vi "Feedback_ver1.vi"(4 "Default output":T3, 6 "Current Motion":T2, 7 "bound":dbl=10.0, 8 "Iteration":dbl, 9 "Sampled current position":dbl[](array[numeric]), 10 "Current Motion Output":T3, 11 "Initial constants":T4) -> (1 "Rawoffset":dbl[][](array[numeric]), 2 "Updated Motion Output Row":T1)   [LabVIEW 2019]
uses:
  Type_definition_current_motion.ctl
  Type_definition_updated_motion_output_row.ctl
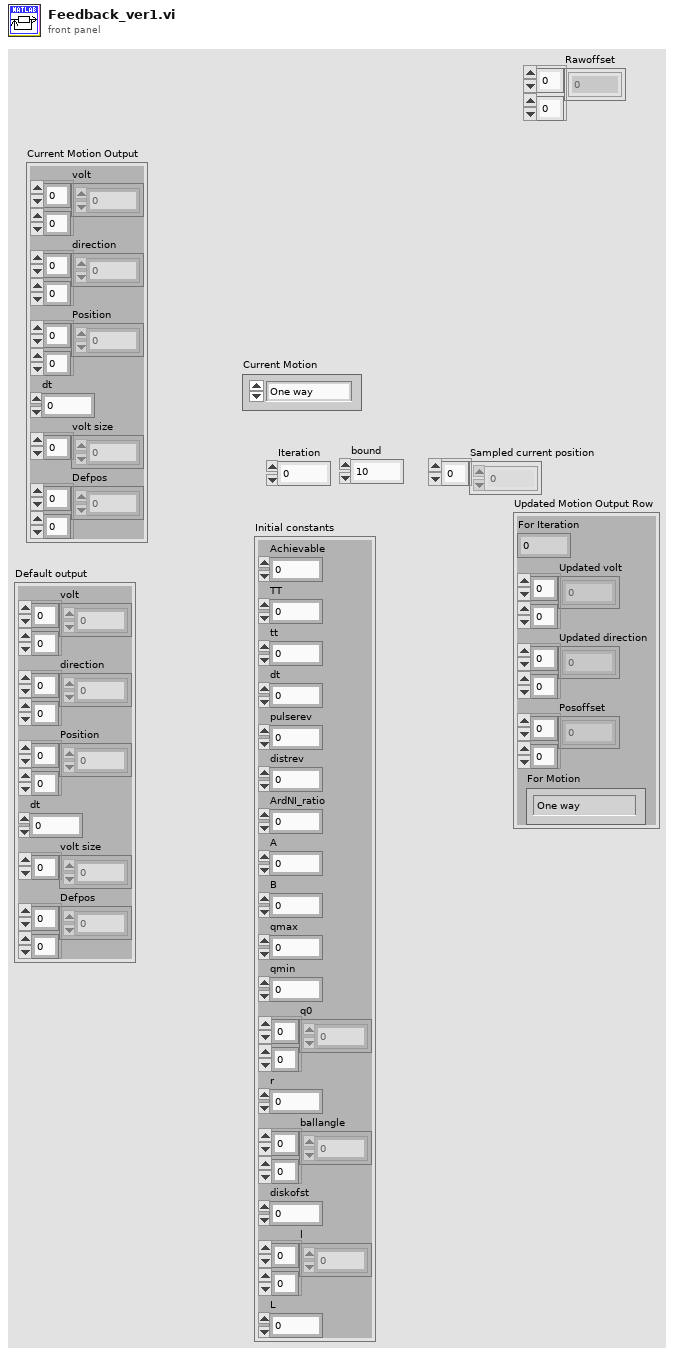
[diagram p1: front panel]
types:
  T1 = typedef "Type_definition_updated_motion_output_row.ctl" = cluster{"For Iteration":dbl, "Updated volt":dbl[][], "Updated direction":dbl[][], "Posoffset":dbl[][], "For Motion":T2}
  T2 = typedef "Type_definition_current_motion.ctl" = enum16{"One way", "Rot", "Tilt", "Tau", "XYZrot", "Zvert", "YZcirc", "Random direction tilt"}
  T3 = cluster{"volt":dbl[][], "direction":dbl[][], "Position":dbl[][], "dt":dbl, "volt size":i32[], "Defpos":dbl[][]}
  T4 = cluster{"Achievable":dbl, "TT":dbl, "tt":dbl, "dt":dbl, "pulserev":dbl, "distrev":dbl, "ArdNI_ratio":dbl, "A":dbl, "B":dbl, "qmax":dbl, "qmin":dbl, "q0":dbl[][], "r":dbl, "ballangle":dbl[][], "diskofst":dbl, "l":dbl[][], "L":dbl}
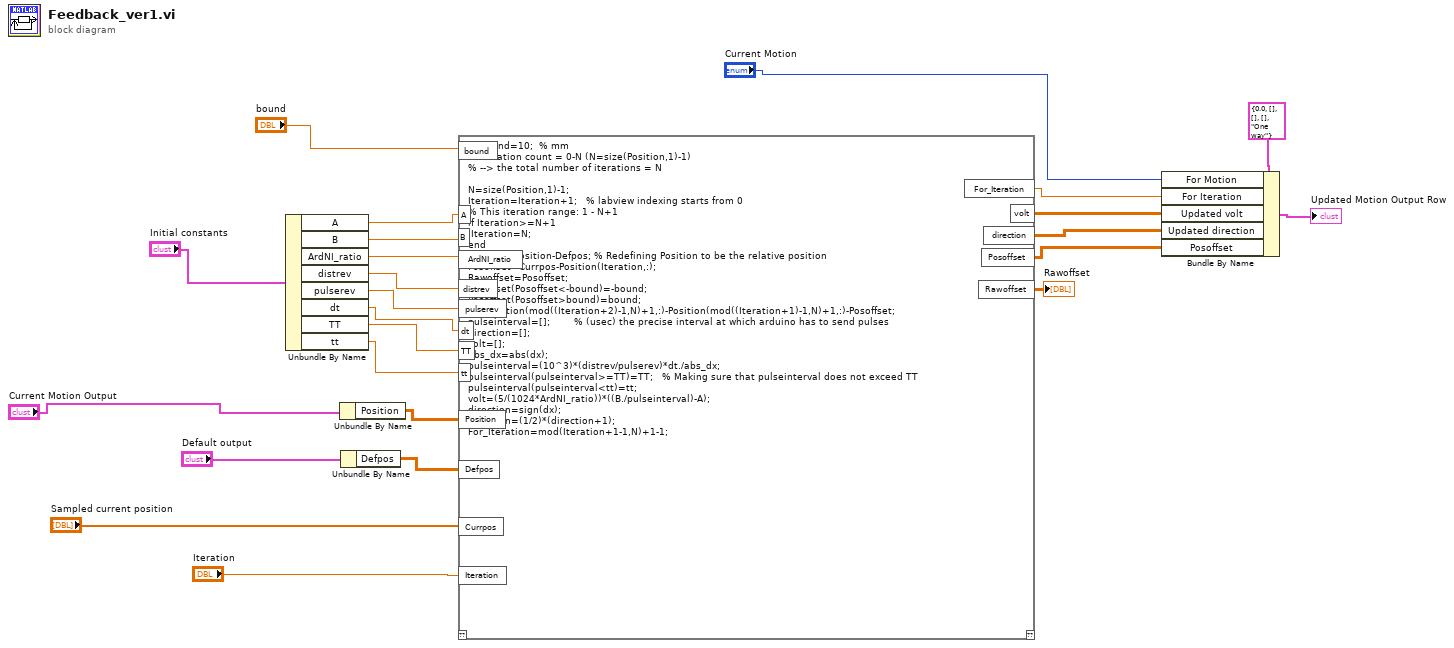
[diagram p0: block diagram]
diagram:
  n1 = Unbundle By Name("Initial constants") -> ("A"=w20:dbl, "B"=w19:dbl, "ArdNI_ratio"=w18:dbl, "distrev"=w17:dbl, "pulserev"=w16:dbl, "dt"=w10:dbl, "TT"=w9:dbl, "tt"=w8:dbl)
  n2 = Unbundle By Name("Current Motion Output") -> ("Position"=w15:dbl[][])
  n3 = Unbundle By Name("Default output") -> ("Defpos"=w7:dbl[][])
  n4 = script code="% bound=10;\t\t% mm\n% Iteration count = 0-N (N=size(Position,1)-1)\n% --> the total number of iterations = N\n\nN=size(Position,1)-1;\nIteration=Iteration+1;\t\t\t% labview indexing starts from 0\n% This iteration range: 1 - N+1\nif Iteration>=N+1\n\tIteration=N;\nend\nPosition=Position-Defpos;\t% Redefining Position to be the relative position\nPosoffset=Currpos-Position(Iteration,:);\nRawoffset=Posoffset;\nPosoffset(Posoffset<-bound)=-bound;\nPosoffset(Posoffset>bound)=bound;\ndx=Position(mod((Iteration+2)-1,N)+1,:)-Position(mod((Iteration+1)-1,N)+1,:)-Posoffset;\npulseinterval=[];\t\t\t\t\t\t\t\t% (usec) the precise interval at which arduino has to send pulses\ndirection=[];\nvolt=[];\nabs_dx=abs(dx);\npulseinterval=(10^3)*(distrev/pulserev)*dt./abs_dx;\npulseinterval(pulseinterval>=TT)=TT;\t\t\t% Making sure that pulseinterval does not exceed TT\npulseinterval(pulseinterval<tt)=tt;\nvolt=(5/(1024*ArdNI_ratio))*((B./pulseinterval)-A);\ndirection=sign(dx);\ndirection=(1/2)*(direction+1);\nFor_Iteration=mod(Iteration+1-1,N)+1-1;"("bound"="bound", "Iteration"="Iteration", "Position"=w15, "Currpos"="Sampled current position", "A"=w20, "B"=w19, "ArdNI_ratio"=w18, "distrev"=w17, "pulserev"=w16, "Defpos"=w7, "dt"=w10, "TT"=w9, "tt"=w8) -> ("volt"=w13:dbl[][], "direction"=w12:dbl[][], "Posoffset"=w11:dbl[][], "For_Iteration"=w14:dbl, "Rawoffset"=→"Rawoffset":dbl[][])  [unwired: 1 in, 1 out]
  n5 = Bundle By Name(cluster=T1 {"For Iteration"=0.0, "Updated volt"=[], "Updated direction"=[], "Posoffset"=[], "For Motion"=enum."One way"} ("Updated Motion Output Row"), "For Motion"="Current Motion", "For Iteration"=w14, "Updated volt"=w13, "Updated direction"=w12, "Posoffset"=w11) -> (→"Updated Motion Output Row":T1)
